vi "Driver_Queue.vi"(0 "Queue N Elements":T2[](array[typedef]), 2 "Queue":T1, 7 "Timeout in ms (0)":i32, 11 "Error In":errorcluster, 13 "Queue Operation":T3) -> (4 "State":string, 6 "Data":variant, 8 "Queue Elements":T2[](array[typedef]), 15 "Error Out":errorcluster)   [LabVIEW 2026, in "Core.lvlib"]
doc: "Queue driver to perform various operations on \"States\" Queue."
uses:
  Core.lvlib
  TypeDefs/Enum_Queue_Options.ctl
  TypeDefs/Cluster_Queue_Element.ctl
  TypeDefs/Enum_Queues.ctl
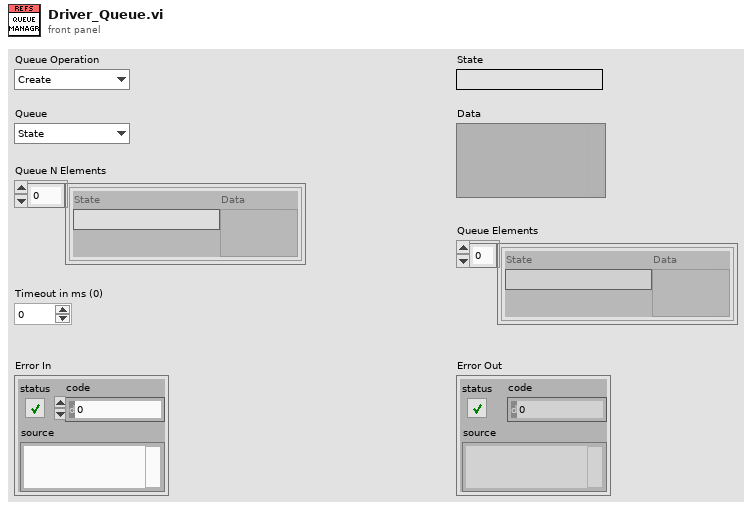
[diagram p1: front panel]
types:
  T1 = typedef "Core.lvlib/Enum_Queues.ctl" = enum16{"State"}
  T2 = typedef "Core.lvlib/Cluster_Queue_Element.ctl" = cluster{"State":string, "Data":variant}
  T3 = typedef "Core.lvlib/Enum_Queue_Options.ctl" = enum16{"Create", "Enqueue N", "Enstack N", "View Queue", "Dequeue", "Flush", "Flush & Close"}
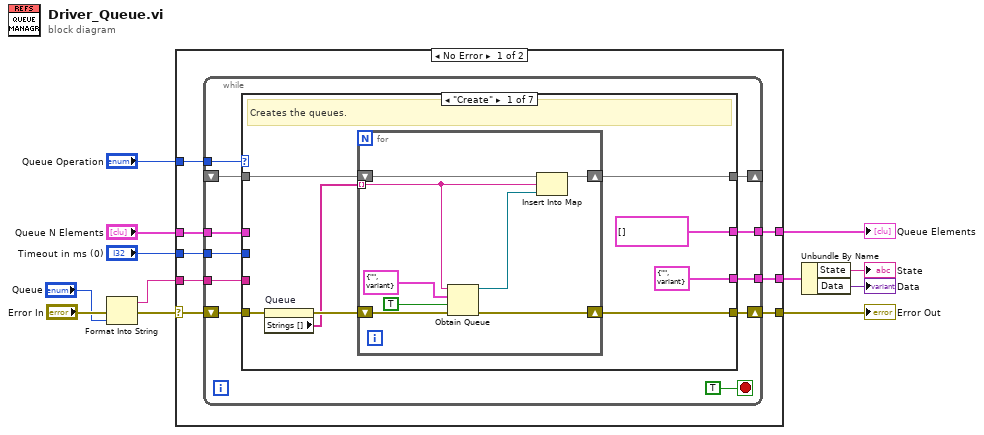
[diagram p0: block diagram]
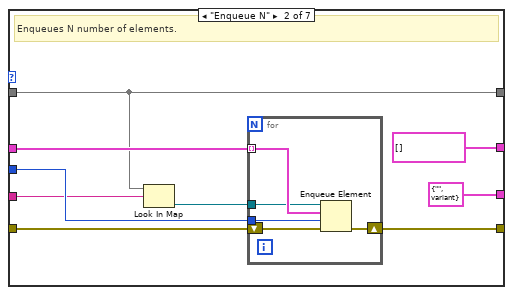
[diagram p2: hidden frame]
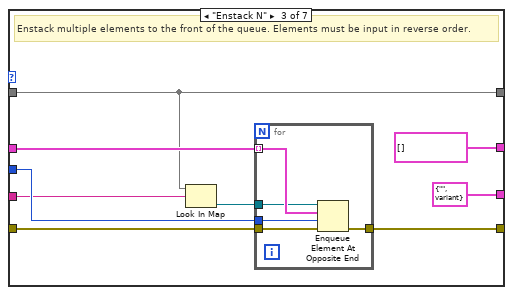
[diagram p3: hidden frame]
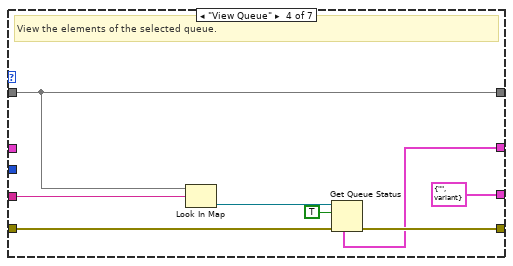
[diagram p4: hidden frame]
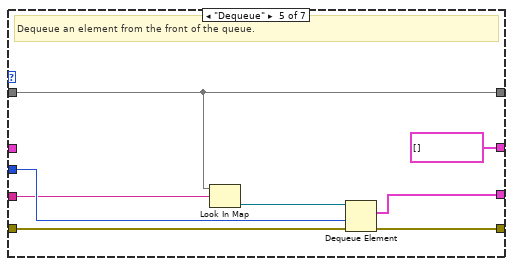
[diagram p5: hidden frame]
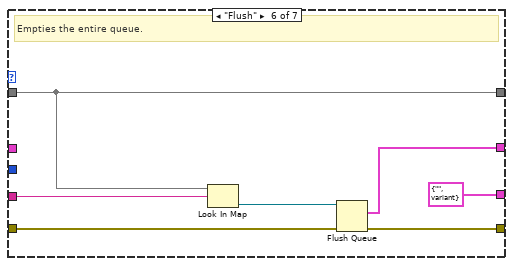
[diagram p6: hidden frame]
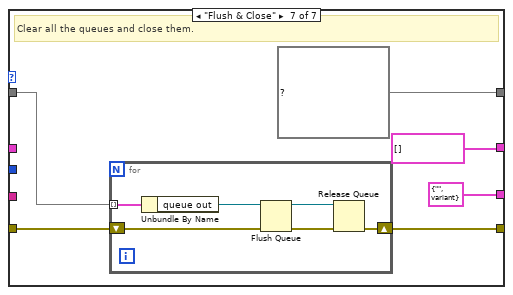
[diagram p7: hidden frame]
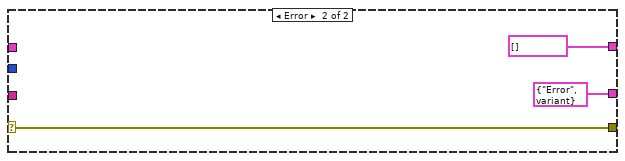
[diagram p8: hidden frame]
diagram:
  n1 = Format Into String(error in="Error In", "Queue") -> (resulting string=w1:string, error out=w3:errorcluster)  [unwired: 2 in]
  n2 = case shown="No Error" w3 {
    selector: w3 -> [w19 w113]
    tunnel: [w18 w113] -> w12
    tunnel: "Queue Operation" -> [w20 _]
    tunnel: "Timeout in ms (0)" -> [w17 _]
    tunnel: [w14 cluster{"State":string, "Data":variant}[] [] ("Queue Elements")] -> w9
    tunnel: "Queue N Elements" -> [w16 _]
    tunnel: [w15 cluster{"State":string, "Data":variant} {"State"="Error", "Data"=variant} ("Queue Element")] -> w7
    tunnel: w1 -> [w13 _]
    frame No Error {
      n3 = while {
        tunnel: w20 -> [w30]
        shift-right: [w29] -> w18
        shift-left: w19 -> [w28]
        tunnel: w17 -> [w27]
        tunnel: w16 -> [w26]
        tunnel: [w25] -> w15
        tunnel: [w24] -> w14
        shift-right: [w21] -> _
        shift-left: _ -> [w22]
        tunnel: w13 -> [w23]
        stop <- TRUE stop-if-true
        n4 = case shown="\"Create\"" w30 {
          tunnel: [w38 w55 w70 w82 w90 w97 w104] -> w29
          tunnel: w28 -> [w39 w56 w69 w83 w91 w98 w103]
          tunnel: w27 -> [_ w54 w68 _ w89 _ _]
          tunnel: w26 -> [_ w52 w66 _ _ _ _]
          tunnel: [T2 {"State"="", "Data"=variant} ("Dequeue Element") T2 {"State"="", "Data"=variant} ("Dequeue Element") T2 {"State"="", "Data"=variant} ("Dequeue Element") T2 {"State"="", "Data"=variant} ("Queue Element") w88 T2 {"State"="", "Data"=variant} ("Queue Element") T2 {"State"="", "Data"=variant} ("Queue Element")] -> w25
          tunnel: [T2[] [] ("Queue Elements") T2[] [] ("Queue Elements") T2[] [] ("Queue Elements") w78 T2[] [] ("Queue Elements") w92 T2[] [] ("Queue Elements")] -> w24
          tunnel: w23 -> [_ w50 w64 w81 w85 w94 _]
          tunnel: w22 -> [w35 w48 w62 w76 w86 w95 w100]
          tunnel: [w34 w48 w62 w76 w86 w95 map{string, refnum<queue>} {} ("map out")] -> w21
          frame "Create" {
            # "Creates the queues."
            n5 = property on="Queue" class="Enum (strict)"(error in=w39) -> (error out=w33:errorcluster, "Strings []"=w32:string[])  [unwired: 1 in, 1 out]
            n6 = for {
              shift-right: [w46] -> w38
              shift-left: w33 -> [w47]
              tunnel: w32 -> [w44] mode=indexing
              shift-right: [w40] -> w34
              shift-left: w35 -> [w41]
              n7 = Obtain Queue(name (unnamed)=w44, element data type=T2 {"State"="", "Data"=variant} ("Queue Element"), create if not found? (T)=TRUE, error in (no error)=w47) -> (queue out=w42:refnum<queue>, error out=w46:errorcluster)  [unwired: 1 in, 1 out]
              n8 = Insert Into Map(map in=w41, key=w44, value=w42) -> (map out=w40:map{string, refnum<queue>})  [unwired: 2 out]
            }
          }
          frame "Enqueue N" {
            # "Enqueues N number of elements."
            n9 = Look In Map(map=w48, key=w50) -> (value=w49:refnum<queue>)  [unwired: 1 in, 1 out]
            n10 = for {
              tunnel: w54 -> [w59]
              tunnel: w52 -> [w58] mode=indexing
              shift-right: [w60] -> w55
              shift-left: w56 -> [w61]
              tunnel: w49 -> [w57]
              n11 = Enqueue Element(queue=w57, element=w58, timeout in ms (-1)=w59, error in (no error)=w61) -> (error out=w60:errorcluster)  [unwired: 2 out]
            }
          }
          frame "Enstack N" {
            # "Enstack multiple elements to the front of the queue. Elements must be input in reverse order."
            n12 = Look In Map(map=w62, key=w64) -> (value=w63:refnum<queue>)  [unwired: 1 in, 1 out]
            n13 = for {
              tunnel: w69 -> [w75]
              tunnel: [w74] -> w70
              tunnel: w68 -> [w73]
              tunnel: w66 -> [w72] mode=indexing
              tunnel: w63 -> [w71]
              n14 = Enqueue Element At Opposite End(queue=w71, element=w72, timeout in ms (-1)=w73, error in (no error)=w75) -> (error out=w74:errorcluster)  [unwired: 2 out]
            }
          }
          frame "View Queue" {
            # "View the elements of the selected queue."
            n15 = Look In Map(map=w76, key=w81) -> (value=w80:refnum<queue>)  [unwired: 1 in, 1 out]
            n16 = Get Queue Status(queue=w80, return elements? (F)=TRUE, error in (no error)=w83) -> (error out=w82:errorcluster, elements=w78:T2[])  [unwired: 6 out]
          }
          frame "Dequeue" {
            # "Dequeue an element from the front of the queue."
            n17 = Look In Map(map=w86, key=w85) -> (value=w84:refnum<queue>)  [unwired: 1 in, 1 out]
            n18 = Dequeue Element(queue=w84, timeout in ms (-1)=w89, error in (no error)=w91) -> (element=w88:T2, error out=w90:errorcluster)  [unwired: 2 out]
          }
          frame "Flush" {
            # "Empties the entire queue."
            n19 = Look In Map(map=w95, key=w94) -> (value=w93:refnum<queue>)  [unwired: 1 in, 1 out]
            n20 = Flush Queue(queue=w93, error in (no error)=w98) -> (remaining elements=w92:T2[], error out=w97:errorcluster)  [unwired: 1 out]
          }
          frame "Flush & Close" {
            # "Clear all the queues and close them."
            n21 = for {
              shift-right: [w110] -> w104
              shift-left: w103 -> [w109]
              tunnel: w100 -> [w106] mode=indexing
              n22 = Unbundle By Name(w106) -> ("queue out"=w105:refnum<queue>)
              n23 = Flush Queue(queue=w105, error in (no error)=w109) -> (queue out=w107:refnum<queue>, error out=w108:errorcluster)  [unwired: 1 out]
              n24 = Release Queue(queue=w107, error in (no error)=w108) -> (error out=w110:errorcluster)  [unwired: 1 in, 2 out]
            }
          }
        }
      }
    }
    frame Error {
    }
  }
  "Error Out" <- w12
  "Queue Elements" <- w9
  n25 = Unbundle By Name(w7) -> ("State"=→"State":string, "Data"=→"Data":variant)
